vi "[ex ce] Real-Time Sound Application.vi"() -> ()   [LabVIEW 2021]
doc: "The main purpose of this example is to demonstrate some peculiarities of using CalcExpress in real-time applications. A simple sound application that uses CalcExpress for data processing was taken for the base.\n\nThis example acquires sound from a sound source, processes it with the use of CalcExpress, and plays resulting sound on an output sound device. Either an input sound device or a wave file can be used as sound source. In both cases, a sound source brings data by portions (data blocks). Data exchange between VIs and scripts is performing through VarMan variables.\n\n::: CalcExpress Toolkit :::\nCopyright (c) 2000-2026 Konstantin Shifershteyn. All rights reserved."
uses:
  <vilib>/sound2/lvsound2.llb/Sound Input Task ID.ctl
panel:
  out "in work":bool
  in  "exit":bool
  in  "stop":bool
  in  "play":bool
  in  "script selector":i32(ring) items=["***  Click here to select an example script  ***", "1. Sound volume control", "2. Adding echo to source sound", "3. Mixing source sound and a background sound", "4. Five-band filtration"]
  in  "expression":string="/*\nThe main purpose of this example is to demonstrate some peculiarities of using CalcExpress in real-time applications. A simple sound application that uses CalcExpress for data processing was taken for the base.\n\nThis example acquires sound from a sound sources, processes it with the use of CalcExpress, and plays resulting sound on an output sound device. Either an input sound device or a wave file can be used as sound source. In both cases, a sound source brings data by portions (blocks). \n\nData exchange between VIs and scripts is performing through predefined variables. The following predefined variables are used in the example:\n\nin - Input data. Data acquired from a sound source is passed to this variable before every script execution. This variable has type 1D Array of DBL.\n\nNs - Buffer size (samples). It has the same value as 'buffer size' control on the Front Panel. Value of this variable is equal to array size of 'in'.\n\nrate - Sampling frequency (Hz). It has the same value as 'Sound Rate' control on the Front Panel.\n\nout - Output data. A value of this variable is passed to output sound device after each execution of script. Note that if 'out' is not changed in a script it saves the previous value. This variable has type 1D Array of DBL.\n*/\n"
  in  "cyclic playing":bool=TRUE
  in  "sel file":bool
  in  "Input Sound device":i32
  in  "Output Sound device":i32
  in  "wave file":path=path "labview.wav"
  in  "Sound Rate : rate":enum16{"11025", "22050", "44100"}(ring)
  in  "buffer size (samples) : Ns":u32=8192 min=1024 step=1024
  in  "Input Sound source":enum16{"wave file", "Sound device"}(ring)
  # "Run the VI, select an example\nscript and click Play button"
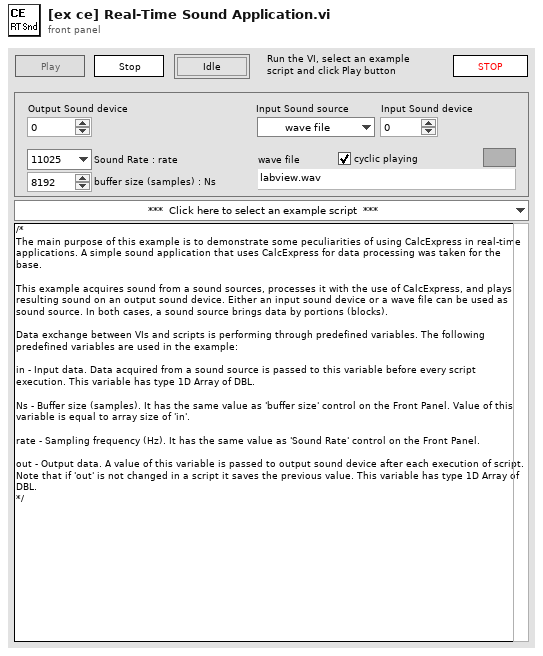
[diagram p1: front panel]
types:
  T1 = typedef "Sound Input Task ID.ctl" = u32
  T2 = typedef "VarMan Variable Context Handle.ctl" = i32
  T3 = typedef "Sound Output Task ID.ctl" = u32
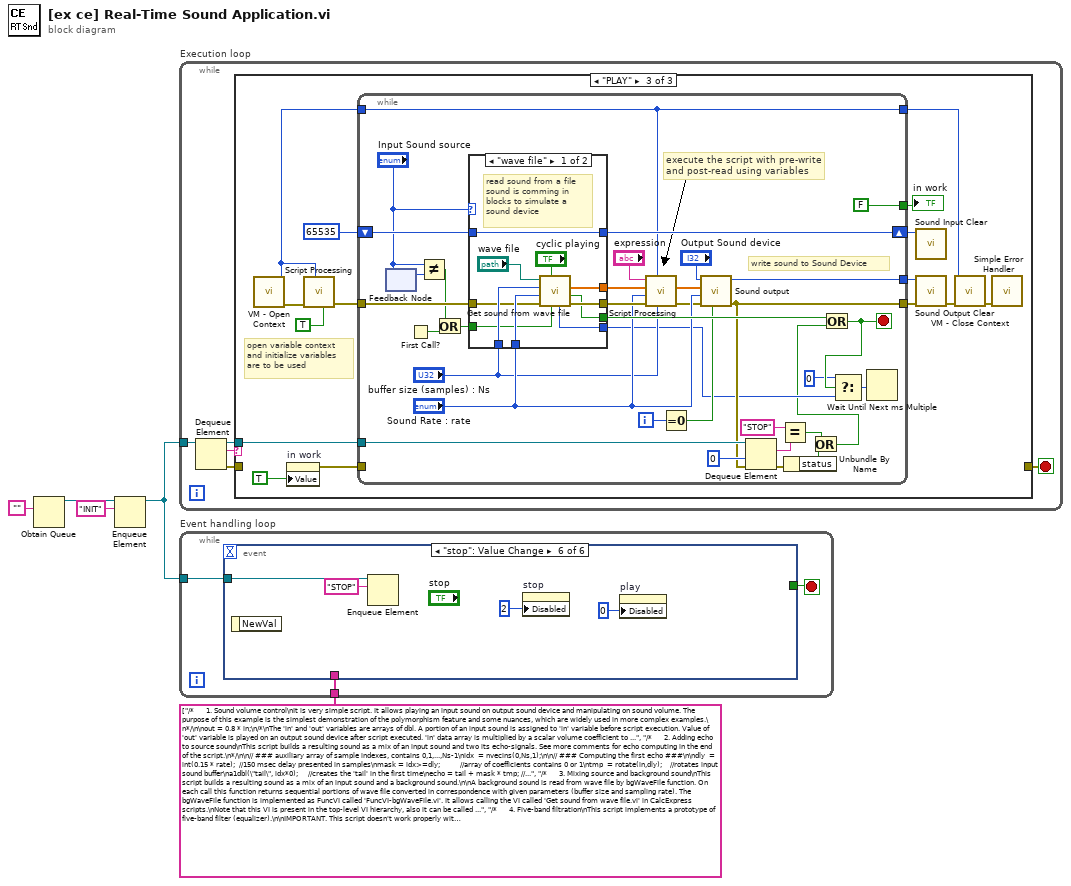
[diagram p0: block diagram]
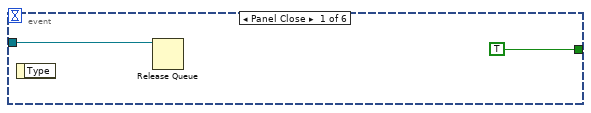
[diagram p2: hidden frame]
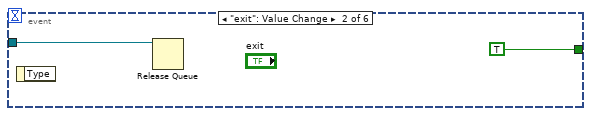
[diagram p3: hidden frame]
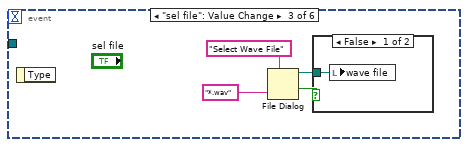
[diagram p4: hidden frame]
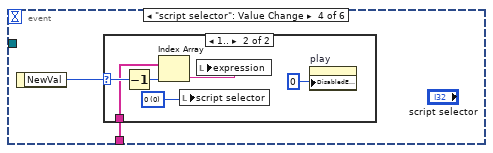
[diagram p6: hidden frame]
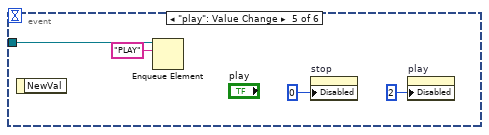
[diagram p8: hidden frame]
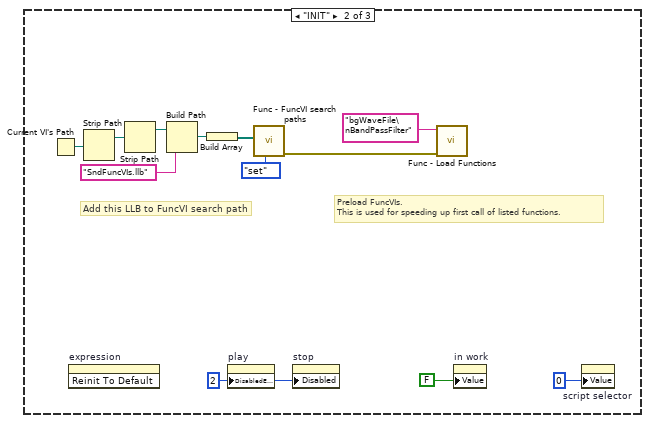
[diagram p10: hidden frame]
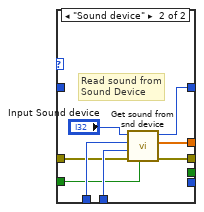
[diagram p11: hidden frame]
diagram:
  n1 = Obtain Queue(element data type="") -> (queue out=w3:refnum<queue>)  [unwired: 4 in, 2 out]
  n2 = Enqueue Element(queue=w3, element="INIT") -> (queue out=w2:refnum<queue>)  [unwired: 2 in, 2 out]
  n3 = while "Execution loop" {
    tunnel: w2 -> [w10]
    stop <- w8 stop-if-true
    n4 = Dequeue Element(queue=w10) -> (queue out=w6:refnum<queue>, element=w9:string, error out=w7:errorcluster)  [unwired: 2 in, 1 out]
    n5 = case shown="\"PLAY\"" w9 {
      tunnel: [w11 _ _] -> w8
      tunnel: w7 -> [w11 _ _]
      tunnel: w6 -> [_ _ w29]
      frame Default {
      }
      frame "INIT" {
        w12 = u8 2
        # "Preload FuncVIs.\nThis is used for speeding up first call of listed functions."
        # "Add this LLB to FuncVI search path"
        n6 = Current VI's Path() -> (path=w19:path)
        n7 = invoke on="expression" class="Str" method="Reinit To Default"() -> ()  [unwired: 3 in, 3 out]
        n8 = Strip Path(path=w19) -> (stripped path=w20:path)  [unwired: 1 out]
        n9 = Strip Path(path=w20) -> (stripped path=w21:path)  [unwired: 1 out]
        n10 = Build Path(base path=w21, name or relative path="SndFuncVIs.llb") -> (appended path=w23:path)
        n11 = Build Array(w23) -> (w16:path[])
        n12 = property on="play" class="Bool"("DisabledEnum"=w12) -> ()  [unwired: 2 in, 2 out]
        n13 = call "Func - FuncVI search paths.vi"("cmd"=enum16{"get", "set"}."set", "user paths"=w16) -> ("error out"=w18:errorcluster)  [unwired: 4 in, 3 out]
        n14 = property on="stop" class="Bool"("Disabled"=w12) -> ()  [unwired: 2 in, 2 out]
        n15 = call "Func - Load Functions.vi"("error in"=w18, "List of func names"="bgWaveFile\nBandPassFilter") -> ()  [unwired: 5 in, 3 out]
        n16 = property on="in work" class="Bool (strict)"("Value"=FALSE ("in work")) -> ()  [unwired: 2 in, 2 out]
        n17 = property on="script selector" class="Ring (strict)"("Value"=0) -> ()  [unwired: 2 in, 2 out]
      }
      frame "PLAY" {
        # "open variable context\nand initialize variables\nare to be used"
        n18 = call "VM - Open Context.vi"() -> ("error out"=w34:errorcluster, "VC Handle out"=w36:T2)  [unwired: 9 in, 1 out]
        n19 = property on="in work" class="Bool (strict)"("Value"=TRUE ("in work")) -> (error out=w28:errorcluster)  [unwired: 2 in, 1 out]
        n20 = call "Script Processing.vi"("init"=TRUE, "VC Handle"=w36, "error in"=w34) -> ("error out"=w38:errorcluster)  [unwired: 6 in, 2 out]
        n21 = while {
          tunnel: w36 -> [w60]
          tunnel: [w60] -> w35
          tunnel: w38 -> [w61]
          shift-left: T1 65535 ("task ID") -> [w69]
          shift-right: [w70] -> w26
          tunnel: [w72] -> w25
          tunnel: [w52] -> w24
          tunnel: [FALSE] -> w30
          tunnel: w29 -> [w53]
          tunnel: w28 -> [_]
          i -> [w57]
          stop <- w58 stop-if-true
          # "write sound to Sound Device"
          # "execute the script with pre-write\nand post-read using variables"
          n22 = feedback #1() -> (w43:enum16{"wave file", "Sound device"})  [unwired: 1 in]
          n23 = feedback-in #1("Input Sound source") -> ()
          n24 = First Call?() -> (First Call?: T/F=w40:bool)
          n25 = Not Equal?(x="Input Sound source", y=w43) -> (x != y?=w39:bool)
          n26 = Or(x=w39, y=w40) -> (x .or. y?=w41:bool)
          n27 = case shown="\"wave file\"" "Input Sound source" {
            tunnel: [w84 w92] -> w68
            tunnel: [w83 w91] -> w67
            tunnel: "Sound Rate : rate" -> [w81 w90]
            tunnel: "buffer size (samples) : Ns" -> [w80 w89]
            tunnel: [w79 _] -> w71
            tunnel: [w77 w87] -> w70
            tunnel: w69 -> [w77 _]
            tunnel: w41 -> [w76 w86]
            tunnel: w61 -> [w75 w85]
            tunnel: [w74 _] -> w45
            frame "wave file" {
              # "read sound from a file\nsound is comming in\nblocks to simulate a\nsound device"
              n28 = call "Get sound from wave file.vi"("init"=w76, "cyclic playing"="cyclic playing", "error in"=w75, "Sound Rate"=w81, "buffer size (samples)"=w80, "wave file"="wave file") -> ("error out"=w84:errorcluster, "EOF"=w79:bool, "sound portion"=w83:dbl[], "delay (ms)"=w74:u32)  [unwired: 1 in, 1 out]
            }
            frame "Sound device" {
              # "Read sound from\nSound Device"
              n29 = call "Get sound from snd device.vi"("init"=w86, "error in"=w85, "Sound Rate"=w90, "buffer size (samples) : Ns"=w89, "Input Sound device"="Input Sound device") -> ("error out"=w92:errorcluster, "sound out"=w91:dbl[], "task ID out"=w87:T1)  [unwired: 2 in]
            }
          }
          n30 = call "Script Processing.vi"("buffer size (samples) : Ns"="buffer size (samples) : Ns", "VC Handle"=w60, "error in"=w68, "Sound Rate : rate"="Sound Rate : rate", "data in"=w67, "script"="expression") -> ("error out"=w63:errorcluster, "data out"=w64:dbl[])  [unwired: 3 in, 1 out]
          n31 = Equal To 0?(x=w57) -> (x = 0?=w56:bool)
          n32 = call "Sound output.vi"("init"=w56, "error in"=w63, "Sound Rate : rate"="Sound Rate : rate", "sound in"=w64, "Output Sound device"="Output Sound device") -> ("error out"=w52:errorcluster, "task ID out"=w72:T3)  [unwired: 3 in]
          n33 = Dequeue Element(queue=w53, timeout in ms (-1)=0, error in (no error)=w52) -> (element=w51:string, error out=w49:errorcluster)  [unwired: 2 out]
          n34 = Equal?(x="STOP", y=w51) -> (x = y?=w47:bool)
          n35 = Unbundle By Name(w49) -> ("status"=w48:bool)
          n36 = Or(x=w47, y=w48) -> (x .or. y?=w44:bool)
          n37 = Or(x=w71, y=w44) -> (x .or. y?=w58:bool)
          n38 = Select(t=u32 0 ("f"), s=w58, f=w45) -> (s? t:f=w59:u32)
          n39 = Wait Until Next ms Multiple(millisecond multiple=w59) -> ()  [unwired: 1 out]
        }
        "in work" <- w30
        n40 = call <vilib>:"Sound Input Clear.vi"("task ID"=w26) -> ()  [unwired: 10 in, 1 out]
        n41 = call <vilib>:"Sound Output Clear.vi"("error in (no error)"=w24, "task ID"=w25) -> ("error out"=w33:errorcluster)  [unwired: 9 in]
        n42 = call "VM - Close Context.vi"("error in"=w33, "VC Handle"=w35) -> ("error out"=w32:errorcluster)  [unwired: 8 in, 1 out]
        n43 = call <vilib>:"Simple Error Handler.vi"("error in (no error)"=w32) -> ()  [unwired: 4 in, 5 out]
      }
    }
  }
  n44 = while "Event handling loop" {
    tunnel: w2 -> [w95]
    tunnel: string[] ["/*      1. Sound volume control\nIt is very simple script. It allows playing an input sound on output sound device and manipulating on sound volume. The purpose of this example is the simplest demonstration of the polymorphism feature and some nuances, which are widely used in more complex examples.\n*/\n\nout = 0.8 * in;\n/*\nThe 'in' and 'out' variables are arrays of dbl. A portion of an input sound is assigned to 'in' variable before script execution. Value of 'out' variable is played on an output sound device after script executed. 'in' data array is multiplied by a scalar volume coefficient to compute value of 'out'.\n*/\n", "/*      2. Adding echo to source sound\nThis script builds a resulting sound as a mix of an input sound and two its echo-signals. See more comments for echo computing in the end of the script.\n*/\n\n// ### auxiliary array of sample indexes, contains 0,1,...,Ns-1\nidx  = nvecins(0,Ns,1);\n\n// ### Computing the first echo ###\n\ndly  = int(0.15 * rate);  //150 msec delay presented in samples\nmask = idx>=dly;          //array of coefficients contains 0 or 1\ntmp  = rotate(in,dly);    //rotates input sound buffer\na1dbl(\"tail\", idx*0);     //creates the 'tail' in the first time\necho = tail + mask * tmp; //an echo for the current step\ntail = !mask * tmp;       //a sound remainder for the next step\n\n// ### Computing the second echo ###\n// It's similar to the first echo computing \n\ndly *= 2;       //delay equals doubled delay of the first echo\ntmp  = rotate(in, dly);\nmask = idx>=dly;\na1dbl(\"tail2\", idx*0);\necho2 = tail2 + mask * tmp;\ntail2 = !mask * tmp;\n\n// ### Computing the resulting sound ###\n\nout = 0.6 * (in + 0.7*echo + 0.3*echo2);\n\n/*   =====================================================\n     Comments to the used method of echo-signal computing.\n     Describes operations in the order.\n     =====================================================\n\n1) idx  = nvecins(0,Ns);\n\nThe 'idx' is an auxiliary array that is used as an index pattern to build masks for computing echo signals. Size of this array is equal to number of samples in input daq buffer. A value of each array element is equal to its index. \n\n2) dly  = int(0.15 * rate);\n\nThe 'dly' variable is equal to delay of echo transformed to number of samples. In this case 'dly' value corresponds to a delay time equal to 150 msec\n\n3) tmp  = rotate(in,dly);\n\nThe 'tmp' contains input sound rotated 'dly' elements to right.\n\n4) mask = idx>=dly;\n\nThe 'mask' is auxiliary array that contains coefficients to compute both delayed sound and 'tail' remaining after rotation of input sound. Elements that have indexes less than dly contain zero, all the other elements contain 1.\n\n5) a1dbl(\"tail\", idx*0)\n\nThe a1dbl function creates and assigns the zeros array to variable 'tail' only if the variable is not defined; i.e. at the first time the script executes. Since the second call, this function doesn't change value of 'tail' because the variable already exist. The 'tail' variable is used to store a tail of sound remaining after shifting input sound. The sound remainder is passed between execution iterations through this variable.\n\n6) echo = tail + mask * tmp\n\nComputes an echo-signal and assigns it to 'echo' variable. The echo-signal contains delayed sound of the current acquisition and sound remainder of previous acquisition. This variable is used to compute a resulting sound.\n\n7) tail = !mask * tmp\n\nComputes a sound remainder and assigns it to 'tail' variable. It will be used at the next processing iteration.\n\n*/\n", "/*      3. Mixing source and background sound\nThis script builds a resulting sound as a mix of an input sound and a background sound.\n\nA background sound is read from wave file by bgWaveFile function. On each call this function returns sequential portions of wave file converted in correspondence with given parameters (buffer size and sampling rate). The bgWaveFile function is implemented as FuncVI called 'FuncVI-bgWaveFile.vi'. It allows calling the VI called 'Get sound from wave file.vi' in CalcExpress scripts.\nNote that this VI is present in the top-level VI hierarchy, also it can be called from scripts with the use of this method.\n*/\n\nout  = in + 0.7 * bgWaveFile(\"banjo.wav\", rate, Ns); //mixing\n/*\nNote. Separators in file path has to be present as double backslash because a single backslash character starts a escape sequence in string constants. For sample,\nbgWaveFile(\"c:\\\\winnt\\\\media\\\\ringin.wav\", rate, Ns)\n*/\n\nout *= 0.8;   //volume control\n\n", "/*      4. Five-band filtration\nThis script implements a prototype of five-band filter (equalizer).\n\nIMPORTANT. This script doesn't work properly without Advanced Analysis Package.\n\nThe main peculiarity of implementation of filter functions (FuncVIs) for real time applications is necessity to keep an internal state of filter for each instance to use it in the next call. In this example, the auxiliary variables are used to store filter states. Names of such variables are passed to filter function (FuncVI) as string arguments and have to be unique for each instance. The FuncVI automatically creates (if it's necessary) and uses these variables to store filter states.\n\nThe BPFilterBtw function is made as FuncVI calledd 'FuncVI-BPFilterBtw.vi'. This function (FuncVI) implements the bandpass Butterworth filter and has the following prototype:\n\na1dbl BPFilterBtw( a1dbl  data,\n                   dbl    SamplesFrequency,\n                   dbl    HighFrequency,\n                   dbl    LowFrequency,\n                   dbl    FilterOrder,\n                   str    StateVarName )\n , where a1dbl is 1D Array of Dbl.\nThe function returns filtered data.\n======================================================\n*/\n\nout  = 3.0 * BPFilterBtw(in, rate,  300,   60, 4, \"f1stat\");\nout += 2.0 * BPFilterBtw(in, rate,  600,  300, 4, \"f2stat\");\nout += 1.0 * BPFilterBtw(in, rate, 1200,  600, 4, \"f3stat\");\nout += 1.5 * BPFilterBtw(in, rate, 2400, 1200, 4, \"f4stat\");\nout += 1.8 * BPFilterBtw(in, rate, 5500, 2400, 4, \"f5stat\");\n\nout *= 0.4;  //common volume control\n"] -> [w93]
    stop <- w94 stop-if-true
    n45 = event shown="[5] \"stop\": Value Change" {
      selector: _ -> [_ _ _ _ _ _]
      dyn-events: _ -> [_ _ _ _ _ _]
      timeout: _ -> [_ _ _ _ _ _]
      tunnel: w95 -> [w97 w99 _ _ w114 w118]
      tunnel: [TRUE TRUE _ _ _ _] -> w94
      tunnel: w93 -> [_ _ _ w105 _ _]
      event Panel Close {
        n46 = event-data() -> ()  [unwired: 1 in, 1 out]
        n47 = Release Queue(queue=w97) -> ()  [unwired: 2 in, 3 out]
      }
      event "exit": Value Change {
        n48 = event-data() -> ()  [unwired: 1 in, 1 out]
        n49 = Release Queue(queue=w99) -> ()  [unwired: 2 in, 3 out]
      }
      event "sel file": Value Change {
        n50 = event-data() -> ()  [unwired: 1 in, 1 out]
        n51 = File Dialog(6:"*.wav" ("pattern"), 7:"Select Wave File" ("prompt")) -> (1:w101:bool, 3:w100:path)  [unwired: 5 in, 2 out]
        n52 = case shown="False" w101 {
          tunnel: w100 -> [w104 _]
          frame False {
            n53 = local write "wave file"(w104) -> ()
          }
          frame True {
          }
        }
      }
      event "script selector": Value Change {
        n54 = event-data() -> ("NewVal"=w106:i32)  [unwired: 1 in]
        n55 = case shown="1.." w106 {
          selector: w106 -> [_ w112]
          tunnel: w105 -> [_ w110]
          frame ..0 {
          }
          frame 1.. {
            w108 = u16 0 items=["0", "1. Redirection of input sound to Output Sound Device"] ("script selector")
            n56 = Decrement(x=w112) -> (x-1=w111:i32)
            n57 = Index Array(array=w110, index=w111) -> (element=w109:string)
            n58 = local write "script selector"(w108) -> ()
            n59 = local write "expression"(w109) -> ()
            n60 = property on="play" class="Bool"("DisabledEnum"=u8 0) -> ()  [unwired: 2 in, 2 out]
          }
        }
      }
      event "play": Value Change {
        n61 = event-data() -> ()  [unwired: 1 in, 1 out]
        n62 = Enqueue Element(queue=w114, element="PLAY") -> ()  [unwired: 2 in, 3 out]
        n63 = property on="stop" class="Bool"("Disabled"=u8 0) -> ()  [unwired: 2 in, 2 out]
        n64 = property on="play" class="Bool"("Disabled"=u8 2) -> ()  [unwired: 2 in, 2 out]
      }
      event "stop": Value Change {
        n65 = event-data() -> ()  [unwired: 1 in, 1 out]
        n66 = Enqueue Element(queue=w118, element="STOP") -> ()  [unwired: 2 in, 3 out]
        n67 = property on="stop" class="Bool"("Disabled"=u8 2) -> ()  [unwired: 2 in, 2 out]
        n68 = property on="play" class="Bool"("Disabled"=u8 0) -> ()  [unwired: 2 in, 2 out]
      }
    }
  }
